vi "Get Stop Delay.vi"(7 "fDelay":sgl, 8 "error in (no error)":errorcluster caption="错误输入（无错误）", 9 "nChannel":i32, 10 "nBoard":i32, 11 "nDevId":i32) -> (0 "error out":errorcluster caption="错误输出", 3 "function return":i32, 5 "fDelay out":sgl)   [LabVIEW 2017, in "smncsftmt.lvlib"]
doc: "__declspec(dllexport) int GetStopDelay(int nDevId, int nBoard, int nChannel, float* fDelay);"
uses:
  smncsftmt.lvlib
  smncsftmt.dll
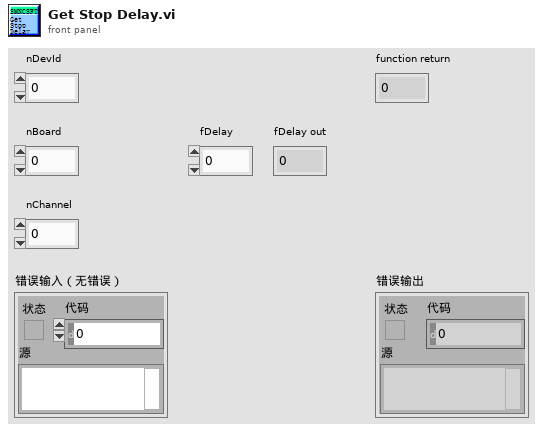
[diagram p1: front panel]
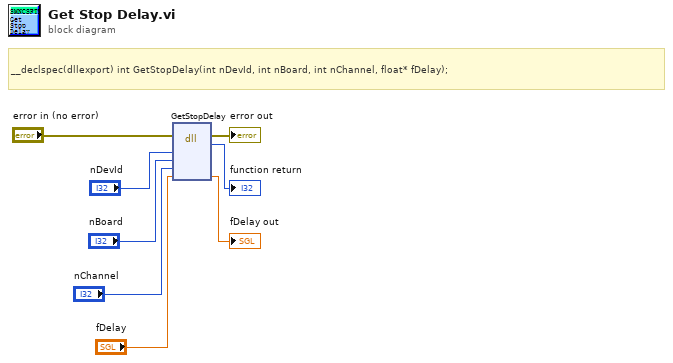
[diagram p0: block diagram]
diagram:
  # "__declspec(dllexport) int GetStopDelay(int nDevId, int nBoard, int nChannel, float* fDelay);"
  n1 = dll-call lib="PTH2oabs CUsersaDesktop\nLABVIEW范例National InstrumentsLabVIEW 2017user.lib\tsmncsftmtsmncsftmt.*" fn="GetStopDelay"(error in="error in (no error)", "nDevId"="nDevId", "nBoard"="nBoard", "nChannel"="nChannel", "fDelay"="fDelay") -> (error out=→"error out":errorcluster, →"function return":i32, "fDelay"=→"fDelay out":sgl)  [unwired: 5 in, 1 out]
